vi "Main.vi"() -> ()   [LabVIEW 2026]
doc: "Use this template to build a simple state machine design pattern. Each state executes code and determines which state to transition to."
uses:
  controls/State.ctl
  controls/Data.ctl
panel:
  out "Saving Data":bool
  out "Vibration History":cluster{"Acceleration":dbl, "vm":dbl}(graph)
  in  "Disturb Mass":bool
  in  "Exit":bool
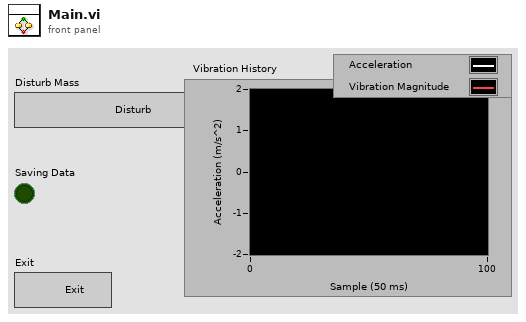
[diagram p1: front panel]
types:
  T1 = typedef "Data.ctl" = cluster{"Settled":bool, "Disturb Time (s)":dbl, "Acceleration":dbl, "File":refnum<file>}
  T2 = typedef "State.ctl" = enum16{"Initialize", "Wait for Event", "Disturb Mass", "Save Data", "Read Data", "Exit"}
  T3 = enum16{"open", "replace", "create", "open or create", "replace or create", "replace or create with confirmation"}
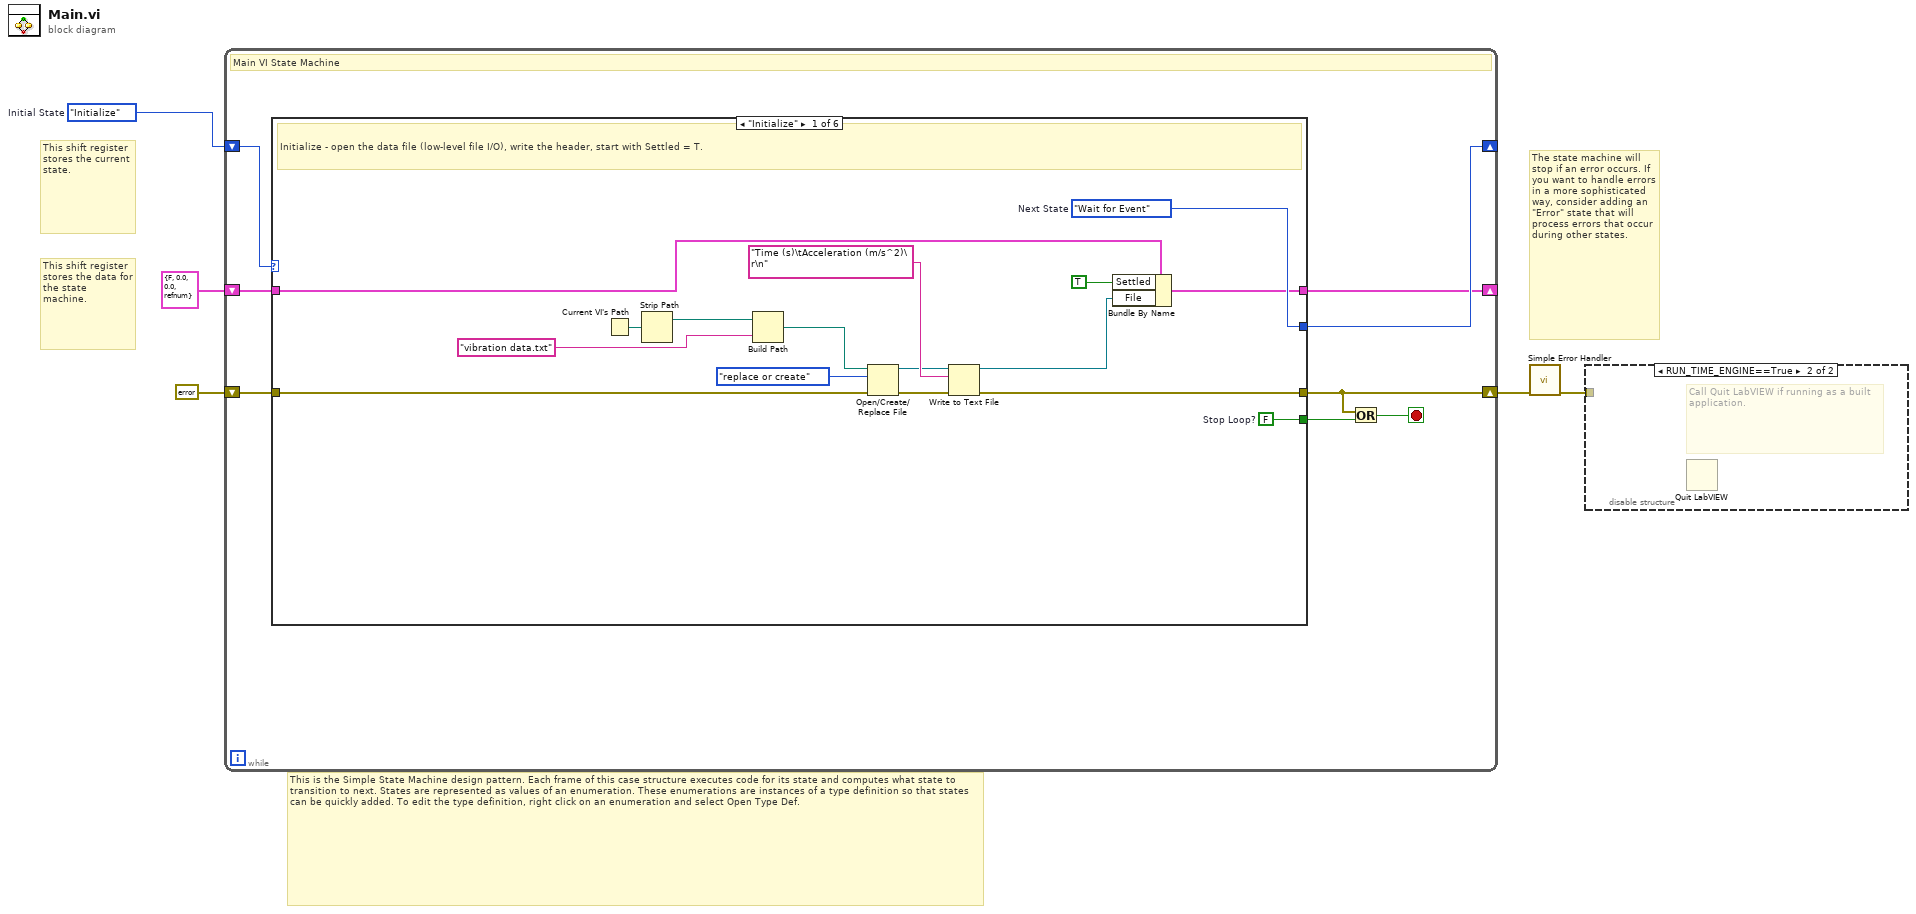
[diagram p0: block diagram]
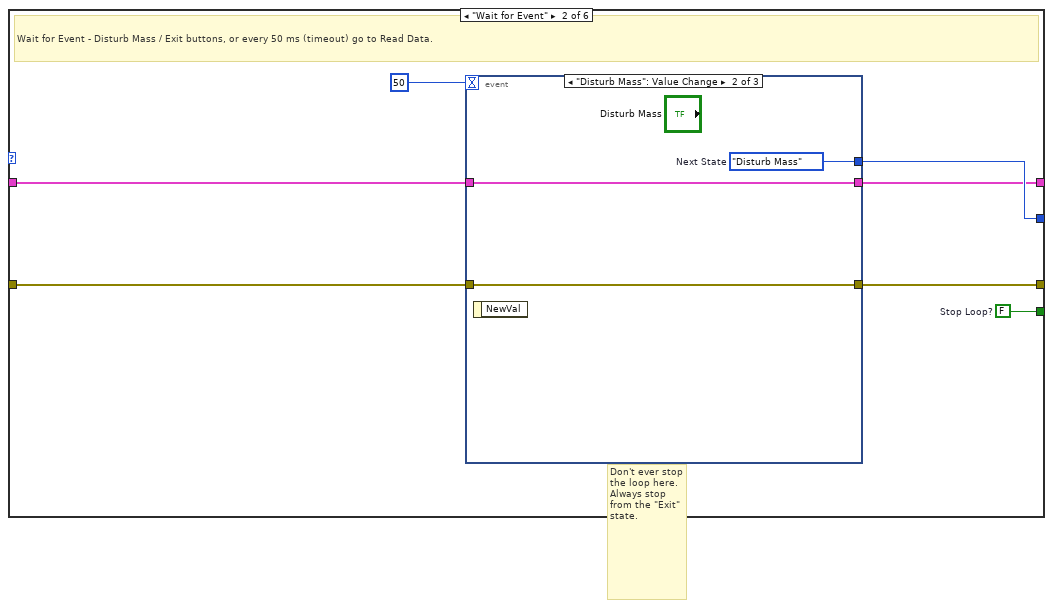
[diagram p3: hidden frame]
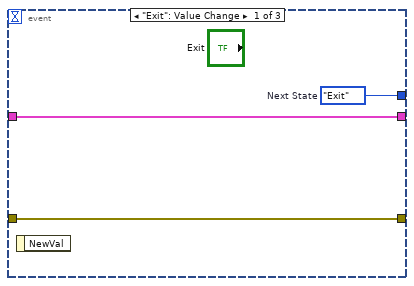
[diagram p4: hidden frame]
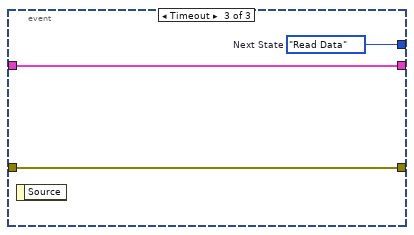
[diagram p5: hidden frame]
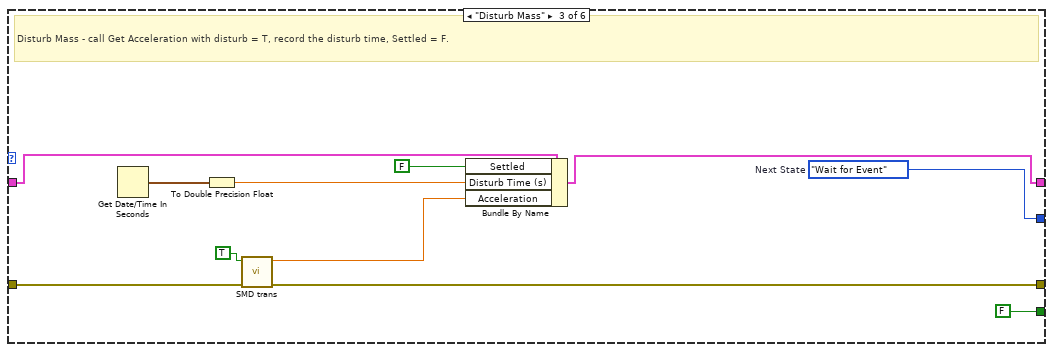
[diagram p6: hidden frame]
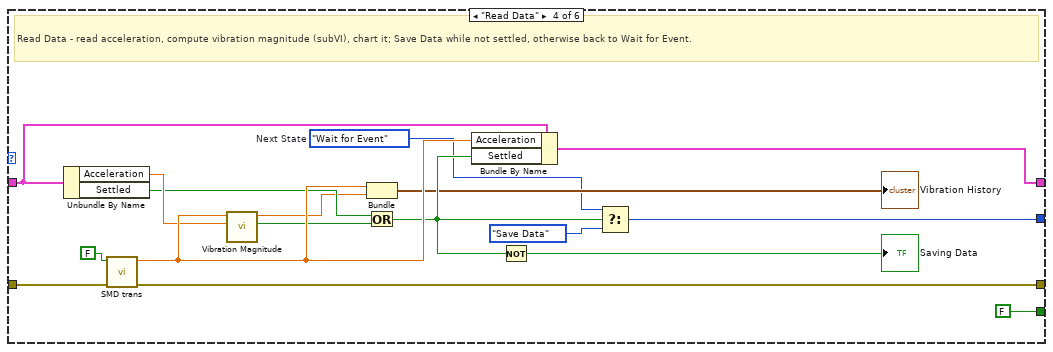
[diagram p7: hidden frame]
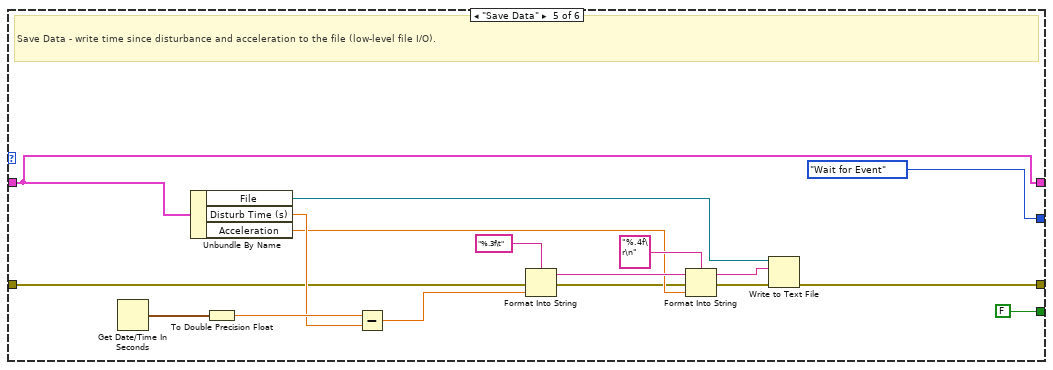
[diagram p8: hidden frame]
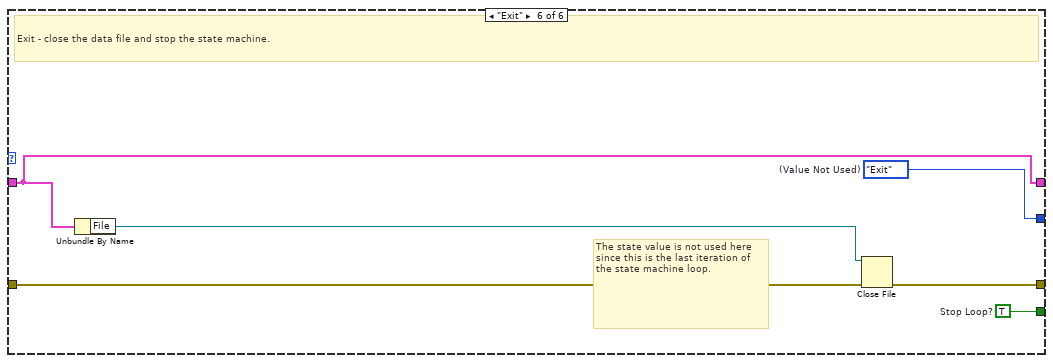
[diagram p9: hidden frame]
diagram:
  w5 = State."Initialize"  # Initial State
  # "The state machine will stop if an error occurs. If you want to handle errors in a more sophisticated way, consider adding an \"Error\" state that will process errors that occur during other states."
  # "This shift register stores the data for the state machine."
  # "This is the Simple State Machine design pattern. Each frame of this case structure executes code for its state and computes what state to transition to next. States are represented as values of an enumeration. These enumerations are instances of a type definition so that states can be quickly added. To edit the type definition, right click on an enumeration and select Open Type Def."
  # "This shift register stores the current state."
  n1 = while {
    shift-right: [w12] -> _
    shift-left: w5 -> [w13]
    shift-right: [w10] -> _
    shift-left: T1 {"Settled"=FALSE, "Disturb Time (s)"=0.0, "Acceleration"=0.0, "File"=refnum} ("Data") -> [w11]
    shift-right: [w6] -> w2
    shift-left: errorcluster {"status"=FALSE, "code"=0, "source"=""} ("error constant") -> [w9]
    stop <- w7 stop-if-true
    # "Main VI State Machine"
    n2 = case shown="\"Initialize\"" w13 {
      tunnel: [w29 w36 w56 w59 State."Wait for Event" ("(Value Not Used)") w96] -> w12
      tunnel: [w28 w35 FALSE ("Stop Loop?") FALSE ("Stop Loop?") FALSE ("Stop Loop?") w94] -> w8
      tunnel: w11 -> [w27 w34 w52 w71 w90 w95]
      tunnel: [w26 w33 w48 w65 w90 w95] -> w10
      tunnel: w9 -> [w17 w32 w47 w58 w79 w92]
      tunnel: [w15 w31 w46 w57 w76 w91] -> w6
      frame "Initialize" {
        w28 = FALSE  # Stop Loop?
        w29 = State."Wait for Event"  # Next State
        # "Initialize - open the data file (low-level file I/O), write the header, start with Settled = T."
        n3 = Current VI's Path() -> (path=w24:path)
        n4 = Strip Path(path=w24) -> (stripped path=w23:path)  [unwired: 1 out]
        n5 = Build Path(base path=w23, name or relative path="vibration data.txt") -> (appended path=w21:path)
        n6 = Open/Create/Replace File(file path (use dialog)=w21, error in=w17, operation (0:open)=T3."replace or create") -> (refnum out=w18:refnum<file>, error out=w16:errorcluster)  [unwired: 3 in, 1 out]
        n7 = Write to Text File(file (use dialog)=w18, text="Time (s)\tAcceleration (m/s^2)\r\n", error in=w16) -> (refnum out=w14:refnum<file>, error out=w15:errorcluster)  [unwired: 1 in, 1 out]
        n8 = Bundle By Name(cluster=w27, "Settled"=TRUE ("Replace_Me_Boolean"), "File"=w14) -> (w26:T1)
      }
      frame "Wait for Event" {
        w35 = FALSE  # Stop Loop?
        # "Don't ever stop the loop here. Always stop from the \"Exit\" state."
        # "Wait for Event - Disturb Mass / Exit buttons, or every 50 ms (timeout) go to Read Data."
        n9 = event shown="[1] \"Disturb Mass\": Value Change" {
          selector: _ -> [_ _ _]
          dyn-events: _ -> [_ _ _]
          timeout: 50 -> [_ _ _]
          tunnel: [w39 w42 w45] -> w36
          tunnel: w34 -> [w38 w40 w43]
          tunnel: [w38 w40 w43] -> w33
          tunnel: w32 -> [w37 w41 w44]
          tunnel: [w37 w41 w44] -> w31
          event "Exit": Value Change {
            w39 = State."Exit"  # Next State
            n10 = event-data() -> ()  [unwired: 1 in, 1 out]
          }
          event "Disturb Mass": Value Change {
            w42 = State."Disturb Mass"  # Next State
            n11 = event-data() -> ()  [unwired: 1 in, 1 out]
          }
          event Timeout {
            w45 = State."Read Data"  # Next State
            n12 = event-data() -> ()  [unwired: 1 in, 1 out]
          }
        }
      }
      frame "Disturb Mass" {
        w56 = State."Wait for Event"  # Next State
        # "Disturb Mass - call Get Acceleration with disturb = T, record the disturb time, Settled = F."
        n13 = Get Date/Time In Seconds() -> (seconds since 1Jan1904=w53:timestamp)
        n14 = To Double Precision Float(number=w53) -> (double precision float=w50:dbl)
        n15 = call "SMD trans.vi"("error in (no error) 2"=w47, "Disturb"=TRUE) -> ("error in (no error) 3"=w46:errorcluster, "Acceleration"=w49:dbl)  [unwired: 8 in]
        n16 = Bundle By Name(cluster=w52, "Settled"=FALSE, "Disturb Time (s)"=w50, "Acceleration"=w49) -> (w48:T1)
      }
      frame "Read Data" {
        w61 = State."Wait for Event"  # Next State
        # "Read Data - read acceleration, compute vibration magnitude (subVI), chart it; Save Data while not settled, otherwise back to Wait for Event."
        n17 = Unbundle By Name(w71) -> ("Acceleration"=w69:dbl, "Settled"=w68:bool)
        n18 = call "SMD trans.vi"("error in (no error) 2"=w58, "Disturb"=FALSE) -> ("error in (no error) 3"=w57:errorcluster, "Acceleration"=w70:dbl)  [unwired: 8 in]
        n19 = call "Vibration Magnitude.vi"("a_n-1"=w69, "a_n"=w70) -> ("Settled (vm<0.1)"=w67:bool, "vm"=w64:dbl)  [unwired: 8 in]
        n20 = Bundle("Acceleration"=w70, "vm"=w64) -> (→"Vibration History":cluster{"Acceleration":dbl, "vm":dbl})  [unwired: 1 in]
        n21 = Or(x=w68, y=w67) -> (x .or. y?=w66:bool)
        n22 = Bundle By Name(cluster=w71, "Acceleration"=w70, "Settled"=w66) -> (w65:T1)
        n23 = Not(x=w66) -> (.not. x?=→"Saving Data":bool)
        n24 = Select(t=w61, s=w66, f=State."Save Data") -> (s? t:f=w59:T2)
      }
      frame "Save Data" {
        # "Save Data - write time since disturbance and acceleration to the file (low-level file I/O)."
        n25 = Get Date/Time In Seconds() -> (seconds since 1Jan1904=w89:timestamp)
        n26 = Unbundle By Name(w90) -> ("File"=w81:refnum<file>, "Disturb Time (s)"=w87:dbl, "Acceleration"=w82:dbl)
        n27 = To Double Precision Float(number=w89) -> (double precision float=w88:dbl)
        n28 = Subtract(x=w88, y=w87) -> (x-y=w85:dbl)
        n29 = Format Into String(format string="%.3f\t", error in=w79, w85) -> (resulting string=w83:string, error out=w78:errorcluster)  [unwired: 1 in]
        n30 = Format Into String(format string="%.4f\r\n", initial string=w83, error in=w78, w82) -> (resulting string=w80:string, error out=w77:errorcluster)
        n31 = Write to Text File(file (use dialog)=w81, text=w80, error in=w77) -> (error out=w76:errorcluster)  [unwired: 1 in, 2 out]
      }
      frame "Exit" {
        w94 = TRUE  # Stop Loop?
        w96 = State."Exit"  # (Value Not Used)
        # "The state value is not used here since this is the last iteration of the state machine loop."
        # "Exit - close the data file and stop the state machine."
        n32 = Unbundle By Name(w95) -> ("File"=w93:refnum<file>)
        n33 = Close File(refnum=w93, error in=w92) -> (error out=w91:errorcluster)  [unwired: 1 out]
      }
    }
    n34 = Or(x=w6, y=w8) -> (x .or. y?=w7:bool)
  }
  n35 = call <vilib>:"Simple Error Handler.vi"("error in (no error)"=w2) -> ("error out"=w1:errorcluster)  [unwired: 4 in, 4 out]
  n36 = disable-structure shown="RUN_TIME_ENGINE==True" {
    disable-tunnel: w1 -> [_ _]
    frame condition #0 (active) {
    }
    frame condition #1 {
      # "Call Quit LabVIEW if running as a built application."
      n37 = Quit LabVIEW() -> ()  [unwired: 1 in]
    }
  }
